vi "十字路口仿真V3.1.vi"() -> ()   [LabVIEW 2014]
panel:
  out "PW_N_R":bool
  out "PW_S_R":bool
  out "PW_E_R":bool
  out "PW_W_R":bool
  out "PW_N_G":bool
  out "PW_S_G":bool
  out "PW_E_G":bool
  out "PW_W_G":bool
  out "BK_NS_TH_R":bool
  out "BK_NS_LT_R":bool
  out "BK_EW_TH_R":bool
  out "BK_EW_LT_R":bool
  out "BK_NS_TH_G":bool
  out "BK_NS_LT_G":bool
  out "BK_EW_TH_G":bool
  out "BK_EW_LT_G":bool
  out "loop_count":dbl
  in  "停止":bool
  in  "step_ms":dbl
  out "slice_name":string
  out "cycle_no":dbl
  out "remain_s":dbl
  out "t_s":dbl
  out "EW_LT_G":bool
  out "EW_TH_G":bool
  out "NS_LT_G":bool
  out "NS_TH_G":bool
  out "EW_LT_Y":bool
  out "EW_TH_Y":bool
  out "NS_LT_Y":bool
  out "NS_TH_Y":bool
  out "EW_LT_R":bool
  out "EW_TH_R":bool
  out "NS_LT_R":bool
  out "NS_TH_R":bool
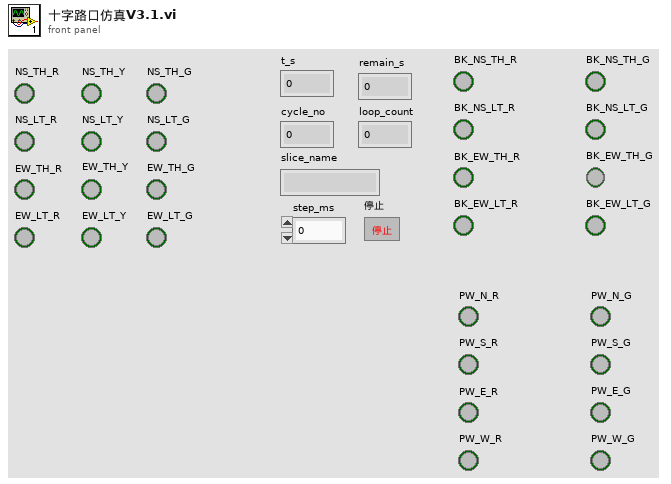
[diagram p1: front panel]
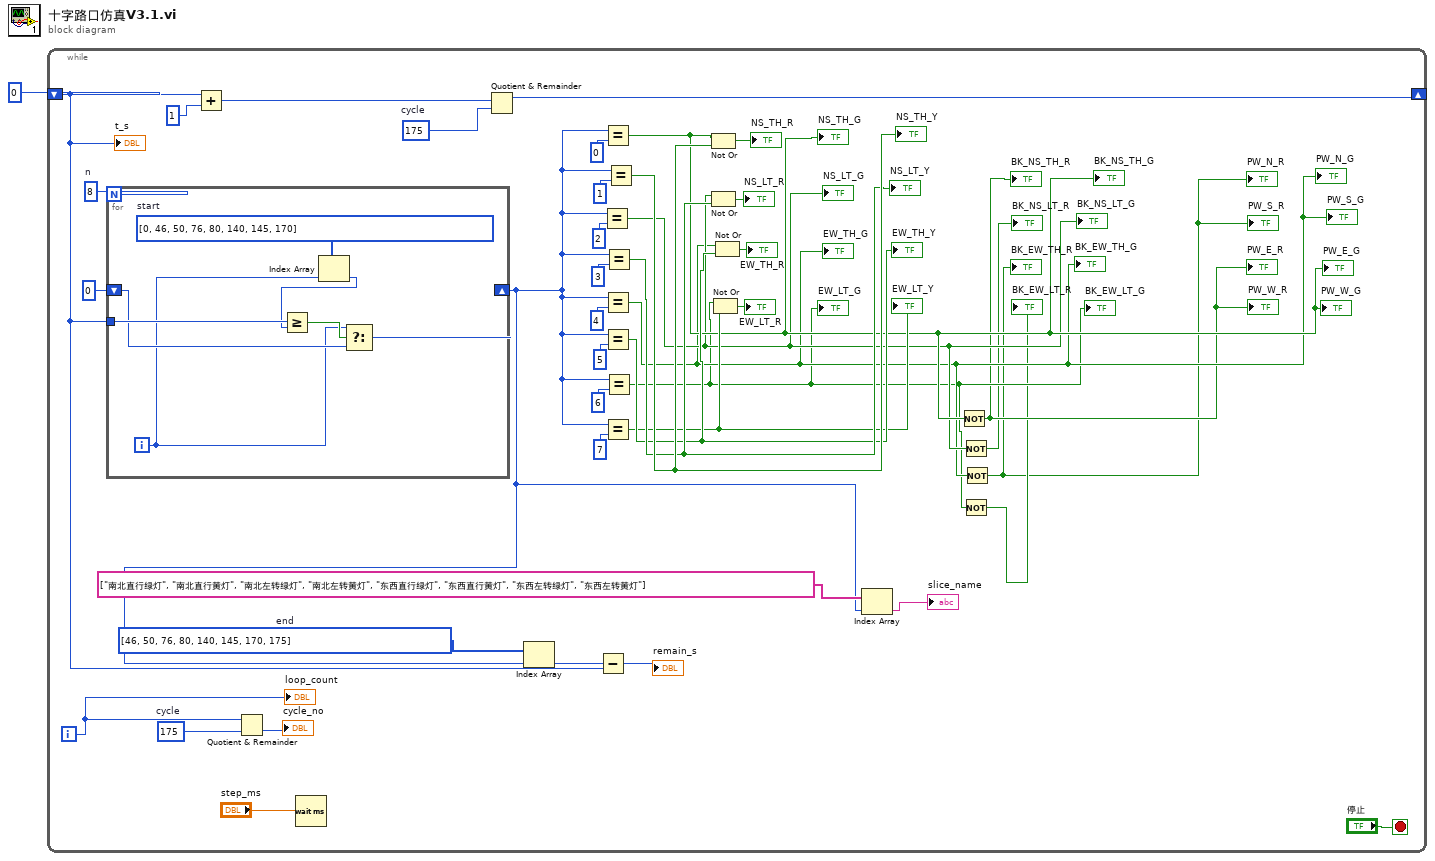
[diagram p0: block diagram]
diagram:
  n1 = while {
    shift-right: [w39] -> _
    shift-left: 0 -> [w31]
    i -> [w28]
    stop <- "停止" stop-if-true
    w30 = 175  # cycle
    w34 = i32[] [46, 50, 76, 80, 140, 145, 170, 175]  # end
    w38 = 8  # n
    w40 = 175  # cycle
    n2 = for {
      N: w38 -> [_]
      shift-right: [w46] -> w18
      shift-left: 0 -> [w47]
      tunnel: w31 -> [w49]
      i -> [w44]
      w50 = i32[] [0, 46, 50, 76, 80, 140, 145, 170]  # start
      n3 = Index Array(array=w50, index=w44) -> (element=w45:i32)
      n4 = Greater Or Equal?(x=w49, y=w45) -> (x >= y?=w48:bool)
      n5 = Select(t=w44, s=w48, f=w47) -> (s? t:f=w46:i32)
    }
    n6 = Add(x=w31, y=1) -> (x+y=w41:i32)
    n7 = Quotient & Remainder(x=w28, y=w30) -> (floor(x/y)=→"cycle_no":i32)  [unwired: 1 out]
    n8 = Wait (ms)(milliseconds to wait="step_ms") -> ()  [unwired: 1 out]
    n9 = Quotient & Remainder(x=w41, y=w40) -> (x-y*floor(x/y)=w39:i32)  [unwired: 1 out]
    n10 = Index Array(array=w34, index=w18) -> (element=w33:i32)
    n11 = Subtract(x=w33, y=w31) -> (x-y=→"remain_s":i32)
    n12 = Equal?(x=w18, y=2) -> (x = y?=w8:bool)
    "NS_LT_G" <- w8
    "BK_NS_LT_G" <- w8
    n13 = Equal?(x=w18, y=0) -> (x = y?=w9:bool)
    "NS_TH_G" <- w9
    "BK_NS_TH_G" <- w9
    "PW_E_G" <- w9
    "PW_W_G" <- w9
    n14 = Equal?(x=w18, y=4) -> (x = y?=w7:bool)
    "EW_TH_G" <- w7
    "BK_EW_TH_G" <- w7
    "PW_N_G" <- w7
    "PW_S_G" <- w7
    n15 = Equal?(x=w18, y=5) -> (x = y?=w11:bool)
    "EW_TH_Y" <- w11
    n16 = Equal?(x=w18, y=7) -> (x = y?=w10:bool)
    "EW_LT_Y" <- w10
    n17 = Equal?(x=w18, y=3) -> (x = y?=w12:bool)
    "NS_LT_Y" <- w12
    n18 = Equal?(x=w18, y=6) -> (x = y?=w6:bool)
    "EW_LT_G" <- w6
    "BK_EW_LT_G" <- w6
    n19 = Equal?(x=w18, y=1) -> (x = y?=w13:bool)
    "NS_TH_Y" <- w13
    n20 = Not Or(1:w13, 2:w9) -> (0:→"NS_TH_R":bool)
    n21 = Not Or(1:w12, 2:w8) -> (0:→"NS_LT_R":bool)
    n22 = Not Or(1:w10, 2:w6) -> (0:→"EW_LT_R":bool)
    n23 = Not Or(1:w11, 2:w7) -> (0:→"EW_TH_R":bool)
    n24 = Index Array(array=string[] ["南北直行绿灯", "南北直行黄灯", "南北左转绿灯", "南北左转黄灯", "东西直行绿灯", "东西直行黄灯", "东西左转绿灯", "东西左转黄灯"], index=w18) -> (element=→"slice_name":string)
    n25 = Not(x=w9) -> (.not. x?=→"BK_NS_TH_R" →"PW_E_R" →"PW_W_R":bool)
    n26 = Not(x=w8) -> (.not. x?=→"BK_NS_LT_R":bool)
    n27 = Not(x=w6) -> (.not. x?=→"BK_EW_LT_R":bool)
    n28 = Not(x=w7) -> (.not. x?=→"BK_EW_TH_R" →"PW_N_R" →"PW_S_R":bool)
    "t_s" <- w31
    "loop_count" <- w28
  }
